vi "M1509DataTrans.vi"(5 "Value":u16[][](array[numeric]), 7 "Meta.Seq":dbl, 9 "Meta.Online":string, 11 "error in":errorcluster) -> (4 "Robot-M1509":T1, 15 "error out":errorcluster)   [LabVIEW 2019]
uses:
  GlobalValue.vi
panel:
  in  "Robot-M1509":T1
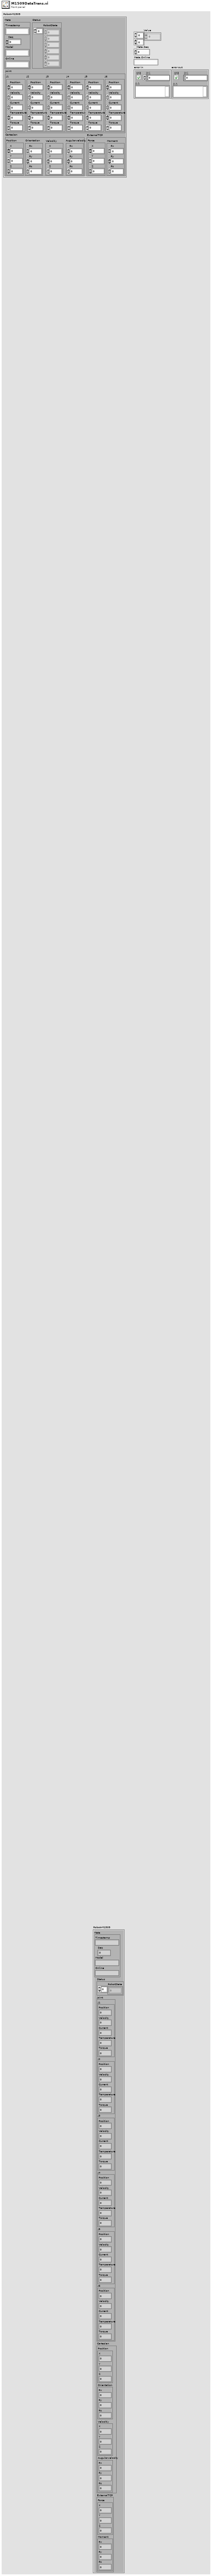
[diagram p1: front panel]
types:
  T1 = cluster{"Meta":cluster{"Timestamp":string, "Seq":dbl, "Model":string, "Online":string}, "Status":cluster{"RobotState":dbl[]}, "Joint":cluster{"J1":cluster{"Position":dbl, "Velocity":dbl, "Current":dbl, "Temperature":dbl, "Torque":dbl}, "J2":cluster{"Position":dbl, "Velocity":dbl, "Current":dbl, "Temperature":dbl, "Torque":dbl}, "J3":cluster{"Position":dbl, "Velocity":dbl, "Current":dbl, "Temperature":dbl, "Torque":dbl}, "J4":cluster{"Position":dbl, "Velocity":dbl, "Current":dbl, "Temperature":dbl, "Torque":dbl}, "J5":cluster{"Position":dbl, "Velocity":dbl, "Current":dbl, "Temperature":dbl, "Torque":dbl}, "J6":cluster{"Position":dbl, "Velocity":dbl, "Current":dbl, "Temperature":dbl, "Torque":dbl}}, "Cartesian":cluster{"Position":cluster{"X":dbl, "Y":dbl, "Z":dbl}, "Orientation":cluster{"Rx":dbl, "Ry":dbl, "Rz":dbl}, "Velocitiy":cluster{"X":dbl, "Y":dbl, "Z":dbl}, "Augularvelocity":cluster{"Rx":dbl, "Ry":dbl, "Rz":dbl}}, "ExternalTCP":cluster{"Force":cluster{"X":dbl, "Y":dbl, "Z":dbl}, "Moment":cluster{"Rx":dbl, "Ry":dbl, "Rz":dbl}}}
  T2 = cluster{"Robot-Delta":cluster{"Meta":cluster{"Timestamp":string, "Seq":dbl, "Model":string, "Online":dbl}, "Status":cluster{"ServoEnabled":dbl, "RobotMotion":string, "ErrorCode":string}, "Joint":cluster{"J13":cluster{"Position":dbl, "Speed":dbl, "Torque":dbl}, "J14":cluster{"Position":dbl, "Speed":dbl, "Torque":dbl}, "J15":cluster{"Position":dbl, "Speed":dbl, "Torque":dbl}}, "Cartesian":cluster{"X":dbl, "Y":dbl, "Z":dbl}}, "Robot-M1509":cluster{"Meta":cluster{"Timestamp":string, "Seq":dbl, "Model":string, "Online":string}, "Status":cluster{"RobotState":dbl[]}, "Joint":cluster{"J1":cluster{"Position":dbl, "Velocity":dbl, "Current":dbl, "Temperature":dbl, "Torque":dbl}, "J2":cluster{"Position":dbl, "Velocity":dbl, "Current":dbl, "Temperature":dbl, "Torque":dbl}, "J3":cluster{"Position":dbl, "Velocity":dbl, "Current":dbl, "Temperature":dbl, "Torque":dbl}, "J4":cluster{"Position":dbl, "Velocity":dbl, "Current":dbl, "Temperature":dbl, "Torque":dbl}, "J5":cluster{"Position":dbl, "Velocity":dbl, "Current":dbl, "Temperature":dbl, "Torque":dbl}, "J6":cluster{"Position":dbl, "Velocity":dbl, "Current":dbl, "Temperature":dbl, "Torque":dbl}}, "Cartesian":cluster{"Position":cluster{"X":dbl, "Y":dbl, "Z":dbl}, "Orientation":cluster{"Rx":dbl, "Ry":dbl, "Rz":dbl}, "Velocitiy":cluster{"X":dbl, "Y":dbl, "Z":dbl}, "Augularvelocity":cluster{"Rx":dbl, "Ry":dbl, "Rz":dbl}}, "ExternalTCP":cluster{"Force":cluster{"X":dbl, "Y":dbl, "Z":dbl}, "Moment":cluster{"Rx":dbl, "Ry":dbl, "Rz":dbl}}}, "Robot-HH7":cluster{"Meta":cluster{"Timestamp":string, "Model":string, "Online":dbl, "Seq":dbl}, "Status":cluster{"RobotMode":dbl, "Playback":dbl, "RemoteMode":dbl, "MotorState":dbl, "EmergencyStop":dbl, "gWaypoint":string}, "Joint":cluster{"J1":cluster{"Position":dbl, "Velocity":dbl, "Torque":dbl}, "J2":cluster{"Position":dbl, "Velocity":dbl, "Torque":dbl}, "J3":cluster{"Position":dbl, "Velocity":dbl, "Torque":dbl}, "J4":cluster{"Position":dbl, "Velocity":dbl, "Torque":dbl}, "J5":cluster{"Position":dbl, "Velocity":dbl, "Torque":dbl}, "J6":cluster{"Position":dbl, "Velocity":dbl, "Torque":dbl}}, "Cartesian":cluster{"Position":cluster{"X":dbl, "Y":dbl, "Z":dbl}, "Orientation":cluster{"Rx":dbl, "Ry":dbl, "Rz":dbl}}, "Errors":cluster{"LastError":string}}, "Robot-AMR":cluster{"Meta":cluster{"Timestamp":string, "Seq":dbl, "Model":string, "Online":dbl}, "LastUpdate":cluster{"Pose":string, "Speed":string, "BaseEncode":string}, "Status":cluster{"NavStatus":dbl, "EmergencyButton":dbl, "ChargeFlag":dbl}, "Pose":cluster{"X":dbl, "Y":dbl, "Theta":dbl}, "Speed":cluster{"Vx":dbl, "Vth":dbl}, "Battery":cluster{"Level":dbl}, "Errors":cluster{"NavStatus":string}}, "Robot-SCARA":cluster{"Meta":cluster{"Timestamp":string, "Model":string, "Seq":dbl, "Online":dbl}, "Status":cluster{"MotorState":dbl, "PowerMode":dbl, "TaskState":dbl, "Waypoint":string}, "Joint":cluster{"J1":cluster{"Position":dbl, "Torque":dbl}, "J2":cluster{"Position":dbl, "Torque":dbl}, "J3":cluster{"Position":dbl, "Torque":dbl}, "J4":cluster{"Position":dbl, "Torque":dbl}}, "Cartesian":cluster{"Position":cluster{"X":dbl, "Y":dbl, "Z":dbl}, "Orientation":cluster{"Rz":dbl}}, "Errors":cluster{"LastError":string}}}
  T3 = cluster{"[0]":dbl, "[1]":dbl, "[2]":dbl, "[3]":dbl, "[4]":dbl, "[5]":dbl, "[6]":dbl, "[7]":dbl, "[8]":dbl}
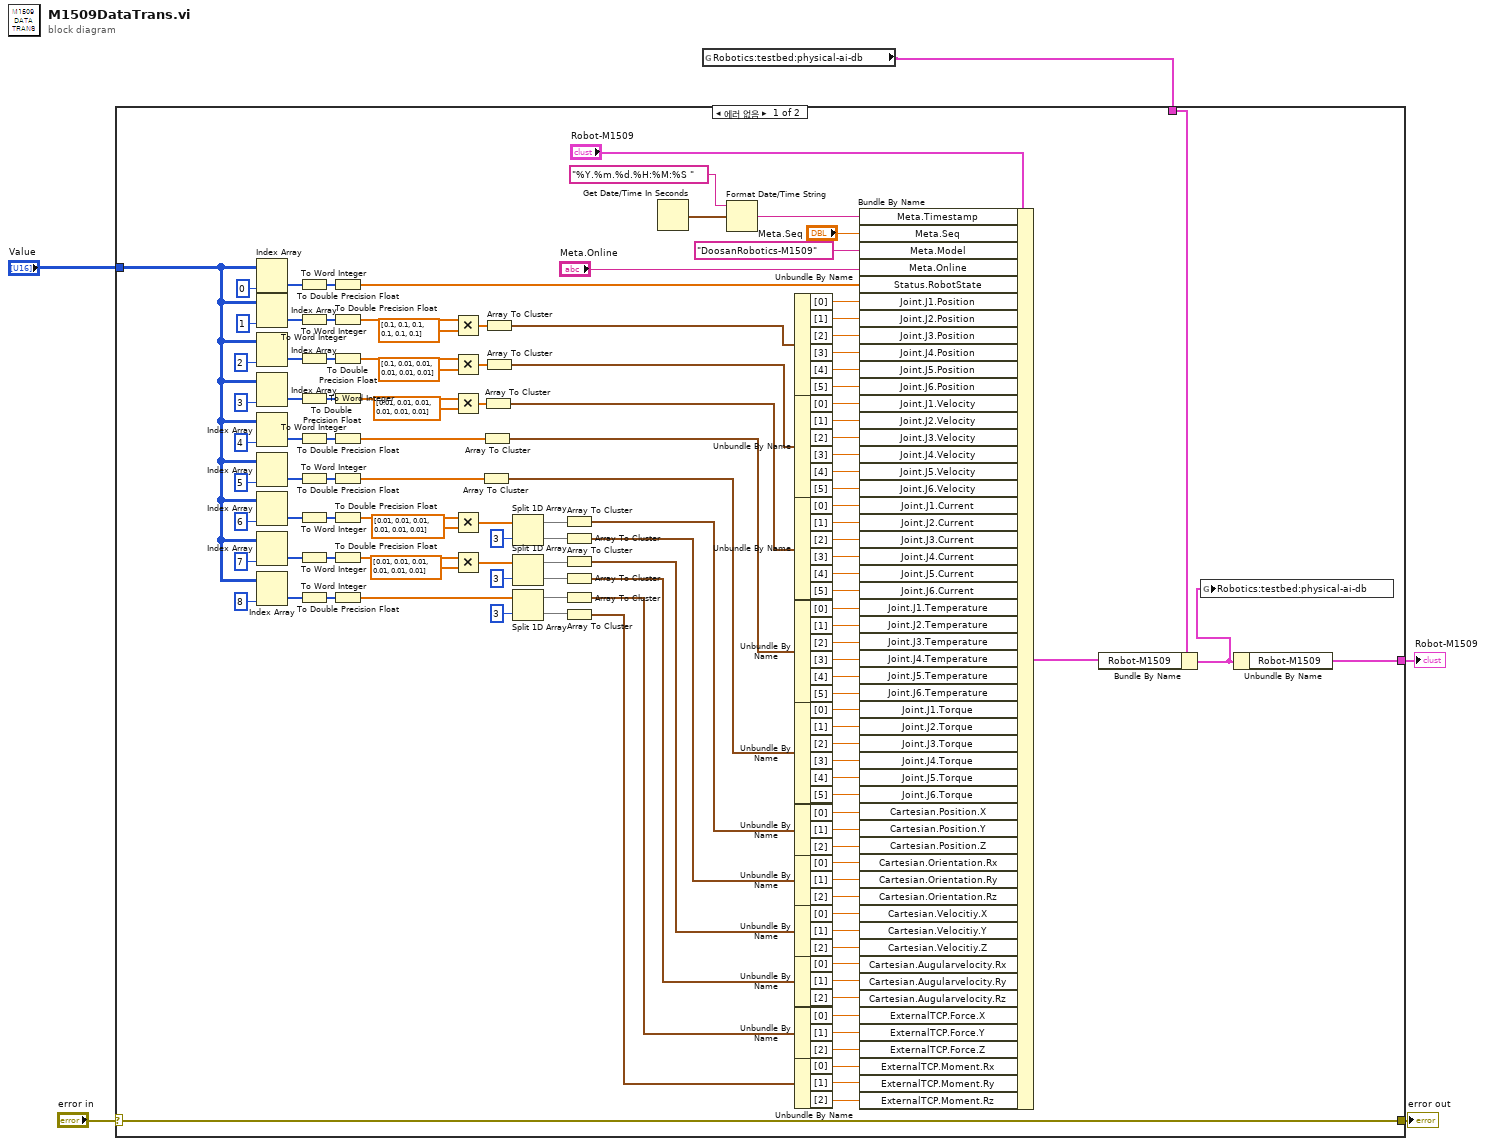
[diagram p0: block diagram]
diagram:
  n1 = global read "GlobalValue.vi" "Robotics:testbed:physical-ai-db"() -> (w2:T2)
  n2 = case shown="에러 없음" "error in" {
    selector: "error in" -> [w12 w133]
    tunnel: "Value" -> [w84 _]
    tunnel: [w12 w133] -> w4
    tunnel: w2 -> [w8 _]
    tunnel: [w9 _] -> w1
    frame No Error {
      n3 = Index Array(array=w84, index (col)=0 ("비활성화된 인덱스 (열)")) -> (element=w90:u16[])  [unwired: 1 in]
      n4 = Index Array(array=w84, index (col)=1 ("비활성화된 인덱스 (열)")) -> (element=w87:u16[])  [unwired: 1 in]
      n5 = Index Array(array=w84, index (col)=2 ("비활성화된 인덱스 (열)")) -> (element=w91:u16[])  [unwired: 1 in]
      n6 = Index Array(array=w84, index (col)=3 ("비활성화된 인덱스 (열)")) -> (element=w94:u16[])  [unwired: 1 in]
      n7 = Index Array(array=w84, index (col)=4 ("비활성화된 인덱스 (열)")) -> (element=w95:u16[])  [unwired: 1 in]
      n8 = Index Array(array=w84, index (col)=5 ("비활성화된 인덱스 (열)")) -> (element=w98:u16[])  [unwired: 1 in]
      n9 = Index Array(array=w84, index (col)=6 ("비활성화된 인덱스 (열)")) -> (element=w103:u16[])  [unwired: 1 in]
      n10 = Index Array(array=w84, index (col)=7 ("비활성화된 인덱스 (열)")) -> (element=w102:u16[])  [unwired: 1 in]
      n11 = Index Array(array=w84, index (col)=8 ("비활성화된 인덱스 (열)")) -> (element=w99:u16[])  [unwired: 1 in]
      n12 = To Word Integer(number=w90) -> (16bit integer=w89:i16[])
      n13 = To Word Integer(number=w87) -> (16bit integer=w88:i16[])
      n14 = To Word Integer(number=w91) -> (16bit integer=w92:i16[])
      n15 = To Word Integer(number=w94) -> (16bit integer=w93:i16[])
      n16 = To Word Integer(number=w95) -> (16bit integer=w96:i16[])
      n17 = To Word Integer(number=w98) -> (16bit integer=w97:i16[])
      n18 = To Word Integer(number=w103) -> (16bit integer=w104:i16[])
      n19 = To Word Integer(number=w102) -> (16bit integer=w101:i16[])
      n20 = To Word Integer(number=w99) -> (16bit integer=w100:i16[])
      n21 = To Double Precision Float(number=w89) -> (double precision float=w83:dbl[])
      n22 = To Double Precision Float(number=w88) -> (double precision float=w113:dbl[])
      n23 = To Double Precision Float(number=w92) -> (double precision float=w115:dbl[])
      n24 = To Double Precision Float(number=w93) -> (double precision float=w117:dbl[])
      n25 = To Double Precision Float(number=w96) -> (double precision float=w58:dbl[])
      n26 = To Double Precision Float(number=w97) -> (double precision float=w57:dbl[])
      n27 = To Double Precision Float(number=w104) -> (double precision float=w119:dbl[])
      n28 = To Double Precision Float(number=w101) -> (double precision float=w121:dbl[])
      n29 = To Double Precision Float(number=w100) -> (double precision float=w126:dbl[])
      n30 = Multiply(x=w113, y=dbl[] [0.1, 0.1, 0.1, 0.1, 0.1, 0.1]) -> (x*y=w82:dbl[])
      n31 = Multiply(x=w115, y=dbl[] [0.1, 0.01, 0.01, 0.01, 0.01, 0.01]) -> (x*y=w74:dbl[])
      n32 = Multiply(x=w117, y=dbl[] [0.01, 0.01, 0.01, 0.01, 0.01, 0.01]) -> (x*y=w66:dbl[])
      n33 = Multiply(x=w119, y=dbl[] [0.01, 0.01, 0.01, 0.01, 0.01, 0.01]) -> (x*y=w122:dbl[])
      n34 = Multiply(x=w121, y=dbl[] [0.01, 0.01, 0.01, 0.01, 0.01, 0.01]) -> (x*y=w125:dbl[])
      n35 = Array To Cluster(array=w57) -> (cluster=w41:T3)
      n36 = Array To Cluster(array=w58) -> (cluster=w48:T3)
      n37 = Array To Cluster(array=w66) -> (cluster=w65:T3)
      n38 = Array To Cluster(array=w82) -> (cluster=w81:T3)
      n39 = Array To Cluster(array=w74) -> (cluster=w73:T3)
      n40 = Split 1D Array(array=w122, index=3 ("인덱스")) -> (first subarray=w56:dbl[], second subarray=w55:dbl[])
      n41 = Split 1D Array(array=w125, index=3 ("인덱스")) -> (first subarray=w31:dbl[], second subarray=w32:dbl[])
      n42 = Split 1D Array(array=w126, index=3 ("인덱스")) -> (first subarray=w30:dbl[], second subarray=w29:dbl[])
      n43 = Array To Cluster(array=w56) -> (cluster=w38:T3)
      n44 = Array To Cluster(array=w55) -> (cluster=w37:T3)
      n45 = Array To Cluster(array=w31) -> (cluster=w16:T3)
      n46 = Array To Cluster(array=w32) -> (cluster=w15:T3)
      n47 = Array To Cluster(array=w30) -> (cluster=w14:T3)
      n48 = Array To Cluster(array=w29) -> (cluster=w13:T3)
      n49 = Get Date/Time In Seconds() -> (seconds since 1Jan1904=w131:timestamp)
      n50 = Format Date/Time String(time format string (%c)="%Y.%m.%d.%H:%M:%S ", seconds (now)=w131) -> (date/time string=w129:string)  [unwired: 1 in]
      n51 = Unbundle By Name(w81) -> ("[0]"=w80:dbl, "[1]"=w79:dbl, "[2]"=w78:dbl, "[3]"=w77:dbl, "[4]"=w76:dbl, "[5]"=w75:dbl)
      n52 = Unbundle By Name(w73) -> ("[0]"=w72:dbl, "[1]"=w71:dbl, "[2]"=w70:dbl, "[3]"=w69:dbl, "[4]"=w68:dbl, "[5]"=w67:dbl)
      n53 = Unbundle By Name(w65) -> ("[0]"=w64:dbl, "[1]"=w63:dbl, "[2]"=w62:dbl, "[3]"=w61:dbl, "[4]"=w60:dbl, "[5]"=w59:dbl)
      n54 = Unbundle By Name(w48) -> ("[0]"=w54:dbl, "[1]"=w53:dbl, "[2]"=w52:dbl, "[3]"=w51:dbl, "[4]"=w50:dbl, "[5]"=w49:dbl)
      n55 = Unbundle By Name(w41) -> ("[0]"=w47:dbl, "[1]"=w46:dbl, "[2]"=w45:dbl, "[3]"=w44:dbl, "[4]"=w43:dbl, "[5]"=w42:dbl)
      n56 = Unbundle By Name(w38) -> ("[0]"=w40:dbl, "[1]"=w33:dbl, "[2]"=w34:dbl)
      n57 = Unbundle By Name(w37) -> ("[0]"=w39:dbl, "[1]"=w35:dbl, "[2]"=w36:dbl)
      n58 = Unbundle By Name(w16) -> ("[0]"=w27:dbl, "[1]"=w26:dbl, "[2]"=w25:dbl)
      n59 = Unbundle By Name(w15) -> ("[0]"=w28:dbl, "[1]"=w24:dbl, "[2]"=w23:dbl)
      n60 = Unbundle By Name(w14) -> ("[0]"=w22:dbl, "[1]"=w21:dbl, "[2]"=w20:dbl)
      n61 = Unbundle By Name(w13) -> ("[0]"=w19:dbl, "[1]"=w18:dbl, "[2]"=w17:dbl)
      n62 = Bundle By Name(cluster="Robot-M1509", "Meta.Timestamp"=w129, "Meta.Seq"="Meta.Seq", "Meta.Model"="DoosanRobotics-M1509", "Meta.Online"="Meta.Online", "Status.RobotState"=w83, "Joint.J1.Position"=w80, "Joint.J2.Position"=w79, "Joint.J3.Position"=w78, "Joint.J4.Position"=w77, "Joint.J5.Position"=w76, "Joint.J6.Position"=w75, "Joint.J1.Velocity"=w72, "Joint.J2.Velocity"=w71, "Joint.J3.Velocity"=w70, "Joint.J4.Velocity"=w69, "Joint.J5.Velocity"=w68, "Joint.J6.Velocity"=w67, "Joint.J1.Current"=w64, "Joint.J2.Current"=w63, "Joint.J3.Current"=w62, "Joint.J4.Current"=w61, "Joint.J5.Current"=w60, "Joint.J6.Current"=w59, "Joint.J1.Temperature"=w54, "Joint.J2.Temperature"=w53, "Joint.J3.Temperature"=w52, "Joint.J4.Temperature"=w51, "Joint.J5.Temperature"=w50, "Joint.J6.Temperature"=w49, "Joint.J1.Torque"=w47, "Joint.J2.Torque"=w46, "Joint.J3.Torque"=w45, "Joint.J4.Torque"=w44, "Joint.J5.Torque"=w43, "Joint.J6.Torque"=w42, "Cartesian.Position.X"=w40, "Cartesian.Position.Y"=w33, "Cartesian.Position.Z"=w34, "Cartesian.Orientation.Rx"=w39, "Cartesian.Orientation.Ry"=w35, "Cartesian.Orientation.Rz"=w36, "Cartesian.Velocitiy.X"=w27, "Cartesian.Velocitiy.Y"=w26, "Cartesian.Velocitiy.Z"=w25, "Cartesian.Augularvelocity.Rx"=w28, "Cartesian.Augularvelocity.Ry"=w24, "Cartesian.Augularvelocity.Rz"=w23, "ExternalTCP.Force.X"=w22, "ExternalTCP.Force.Y"=w21, "ExternalTCP.Force.Z"=w20, "ExternalTCP.Moment.Rx"=w19, "ExternalTCP.Moment.Ry"=w18, "ExternalTCP.Moment.Rz"=w17) -> (w7:T1)
      n63 = Bundle By Name(cluster=w8, "Robot-M1509"=w7) -> (w6:T2)
      n64 = global write "GlobalValue.vi" "Robotics:testbed:physical-ai-db"(w6) -> ()
      n65 = Unbundle By Name(w6) -> ("Robot-M1509"=w9:T1)
    }
    frame Error {
    }
  }
  "error out" <- w4
  "Robot-M1509" <- w1
